vi "WeighBins.vi"(0 "Base Speed":i32, 1 "Cutoff":i32=10, 3 "NXT/EV3 IN":T1, 4 "Tolerance":i32, 5 "Speed Increment":i32=1) -> (2 "IsHeavy":bool, 6 "NXT/EV3 OUT":T1)   [LabVIEW 2016, in "13.03 Robot.lvrbt"]
uses:
  13.03 Robot.lvrbt
  <vilib>/NXT/Subs/LVHSConnector.ctl
  <vilib>/NXT/LegoClasses/BrickReference/BrickReference.lvclass
  <vilib>/NXT/Block Support/NXT_OutputPort.ctl
  <vilib>/NXT/NXTIO Xnodes/NXTIONodeSubVIs/NXTMoveMotors.vi
  <vilib>/NXT/Dual Mode Library/Display/drawNumber.vi
  <vilib>/NXT/NXTIO Xnodes/AddressXNode/NXTIOAddress.xnode
  <vilib>/NXT/NXTIO Xnodes/NXTIOXNode/NXTIO.xnode
panel:
  out "testnum":dbl
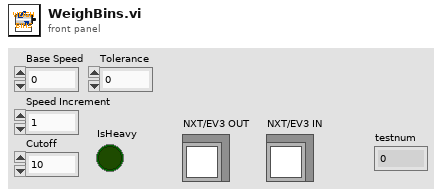
[diagram p1: front panel]
types:
  T1 = typedef "LVHSConnector.ctl" = refnum<class "BrickReference.lvclass">
  T2 = typedef "NXT_OutputPort.ctl" = u8
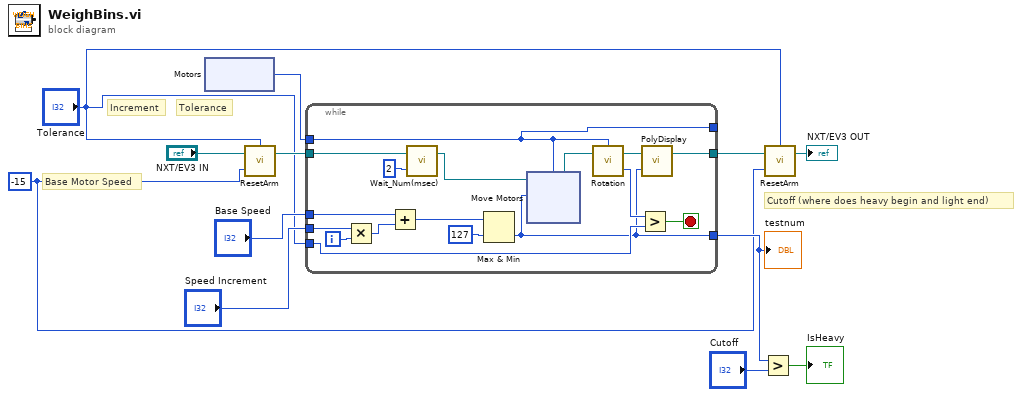
[diagram p0: block diagram]
diagram:
  w4 = i8 -15 ("Power/Speed 1")
  # "Cutoff (where does heavy begin and light end)"
  # "Tolerance"
  # "Increment"
  # "Base Motor Speed"
  n1 = xnode "Motors"() -> ("Motor"=w8:T2)
  n2 = call "ResetArm.vi"("Power/Speed 1"=w4, "NXT/EV3 IN"="NXT/EV3 IN", "ResetTo"="Tolerance") -> ("NXT/EV3 OUT"=w5:T1)
  n3 = while {
    tunnel: "Speed Increment" -> [w28]
    tunnel: "Base Speed" -> [w27]
    tunnel: w8 -> [w24]
    tunnel: "Tolerance" -> [w23]
    tunnel: [w19] -> w3
    tunnel: w5 -> [w15]
    tunnel: [w24] -> _
    tunnel: [w16] -> w7
    i -> [w29]
    stop <- w22 stop-if-true
    n4 = Multiply(x=w28, y=w29) -> (x*y=w26:i32)
    n5 = Add(x=w27, y=w26) -> (x+y=w18:i32)
    n6 = call <vilib>:"Wait_Num(msec).vi"("Time (100 msec)"=u32 2, "NXT/EV3"=w15) -> ("NXT/EV3"=w14:T1)  [unwired: 2 in]
    n7 = Max & Min(x=w18, y=127) -> (min(x,y)=w16:i32)  [unwired: 1 out]
    n8 = xnode "Move Motors"("Power/Speed 1"=w16, "Motors"=w24, "NXT/EV3"=w14) -> ("NXT/EV3"=w25:T1)
    n9 = call <vilib>:"Rotation.vi"("NXT/EV3"=w25, "Port (Port A)"=w24) -> ("Angle of Rotation"=w21:i32, "NXT/EV3"=w20:T1)  [unwired: 1 in]
    n10 = Greater?(x=w21, y=w23) -> (0:w22:bool)
    n11 = call-poly <vilib>:"PolyDisplay.vi"("number"=w16, "NXT/EV3"=w20) -> ("NXT/EV3"=w19:T1)  [unwired: 2 in]
  }
  "testnum" <- w7
  n12 = Greater?(x=w7, y="Cutoff") -> (0:→"IsHeavy":bool)
  n13 = call "ResetArm.vi"("Power/Speed 1"=w4, "NXT/EV3 IN"=w3, "ResetTo"="Tolerance") -> ("NXT/EV3 OUT"=→"NXT/EV3 OUT":T1)
